vi "subSetItemInfoDependencies.vi"(8 "error in (no error)":errorcluster, 11 "SolutionBuilder in":refnum<class "SolutionBuilder.lvclass">) -> (0 "error out":errorcluster, 3 "SolutionBuilder out":refnum<class "SolutionBuilder.lvclass">)   [LabVIEW 2019, in "SolutionBuilder.lvlib" / "SolutionBuilder.lvclass"]
uses:
  SolutionBuilder.lvclass
  NamePathMap.ctl
  SolutionBuilder.lvclass/SolutionBuilder.ctl
  ProjectItem/ProjectItem.lvclass
  SolutionBuilder.lvlib
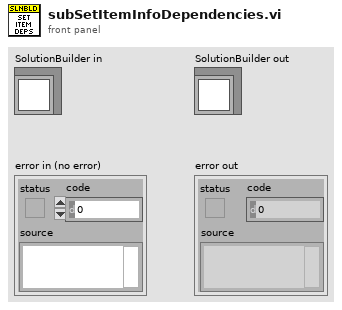
[diagram p1: front panel]
types:
  T1 = typedef "SolutionBuilder.lvlib/SolutionBuilder.lvclass/NamePathMap.ctl" = map{string, path}
  T2 = typedef "SolutionBuilder.lvlib/SolutionBuilder.lvclass/Hashes.ctl" = cluster{"Previous":T3, "Current":T3}
  T3 = typedef "SolutionBuilder.lvlib/SolutionBuilder.lvclass/HashMap.ctl" = map{T4, map{string, string}}
  T4 = typedef "SolutionBuilder.lvlib/SolutionBuilder.lvclass/IncrementalProjectInfo.ctl" = cluster{"Project path":string, "Build spec name":string, "Target":string}
  T5 = typedef "SolutionBuilder.lvlib/SolutionBuilder.lvclass/ProjectItemMap.ctl" = map{path, refnum<class "ProjectItem.lvclass">[]}
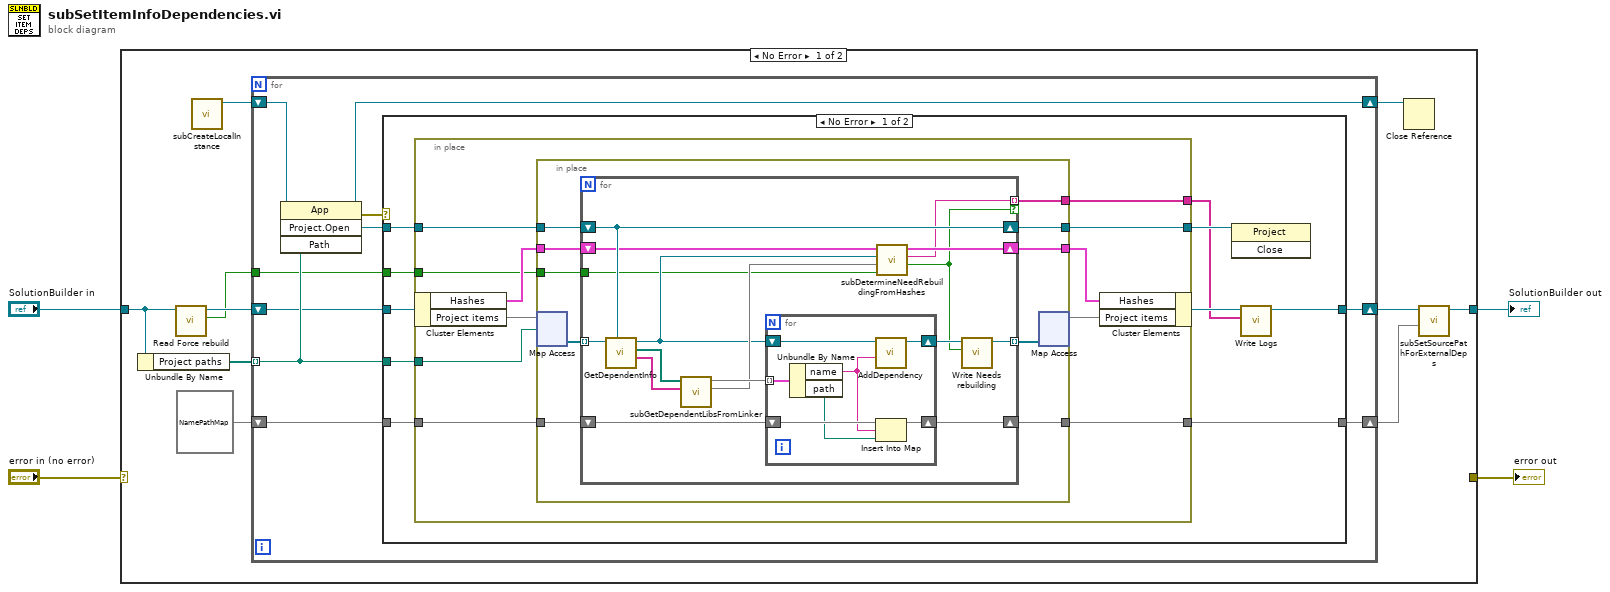
[diagram p0: block diagram]
diagram:
  n1 = case shown="No Error" "error in (no error)" {
    selector: "error in (no error)" -> [_ w81]
    tunnel: [w12 w82] -> w4
    tunnel: "SolutionBuilder in" -> [w7 w82]
    tunnel: [_ w81] -> w1
    frame No Error {
      n2 = Unbundle By Name(w7) -> ("Project paths"=w14:path[])
      n3 = call "Read Force rebuild.vi"("SolutionBuilder in"=w7) -> ("Force rebuild"=w5:bool, "SolutionBuilder out"=w6:refnum<class "SolutionBuilder.lvclass">)  [unwired: 9 in]
      n4 = call "subCreateLocalInstance.vi"() -> ("Application out"=w10:refnum<vi>)  [unwired: 11 in]
      n5 = for {
        tunnel: w14 -> [w22] mode=indexing
        shift-right: [w23] -> w13
        shift-left: T1 {} ("Dependency libs") -> [w24]
        shift-right: [w18] -> w9
        shift-left: w10 -> [w19]
        shift-right: [w16] -> w8
        shift-left: w6 -> [w17]
        tunnel: w5 -> [w15]
        n6 = invoke class="App" method="Project.Open"(reference=w19, "Path"=w22) -> (reference out=w18:refnum<vi>, error out=w21:errorcluster, "Project:Open"=w20:refnum<vi>)  [unwired: 2 in, 1 out]
        n7 = case shown="No Error" w21 {
          tunnel: w24 -> [w34 w80]
          tunnel: [w33 w80] -> w23
          tunnel: w22 -> [w32 _]
          tunnel: w20 -> [w31 _]
          tunnel: w17 -> [w29 w79]
          tunnel: [w27 w79] -> w16
          tunnel: w15 -> [w25 _]
          frame No Error {
            n8 = in-place {
              in-place-border: w34 -> [w45]
              in-place-border: [w44] -> w33
              in-place-border: w32 -> [w43]
              in-place-border: w31 -> [w42]
              in-place-border: [w41] -> w30
              in-place-border: [w36] -> w26
              in-place-border: w25 -> [w35]
              n9 = in-place-cluster #1(w29) -> ("Hashes"=w38:T2, "Project items"=w40:T5)
              n10 = in-place {
                in-place-border: [w53] -> w44
                in-place-border: w45 -> [w52]
                in-place-border: w42 -> [w51]
                in-place-border: [w50] -> w41
                in-place-border: w38 -> [w49]
                in-place-border: [w48] -> w37
                in-place-border: [w47] -> w36
                in-place-border: w35 -> [w46]
                n11 = in-place-map #2(w40, w43) -> (w55:refnum<class "ProjectItem.lvclass">[])  [unwired: 1 in, 1 out]
                n12 = for {
                  tunnel: w55 -> [w67] mode=indexing
                  tunnel: [w63] -> w54 mode=indexing
                  shift-right: [w71] -> w53
                  shift-left: w52 -> [w70]
                  shift-right: [w68] -> w50
                  shift-left: w51 -> [w68]
                  shift-right: [w61] -> w48
                  shift-left: w49 -> [w62]
                  tunnel: [w58] -> w47 mode=indexing if=w57
                  tunnel: w46 -> [w56]
                  n13 = call "GetDependentInfo.vi"("Project ref"=w68, "ProjectItem in"=w67) -> ("Dependent owning libs"=w65:string[], "Dependent paths"=w66:path[], "ProjectItem out"=w59:refnum<class "ProjectItem.lvclass">)  [unwired: 6 in, 1 out]
                  n14 = call "subGetDependentLibsFromLinker.vi"("Owning libs"=w65, "Paths"=w66) -> ("Dependency files"=w60:set{path}, "Dependency libs"=w69:T1)  [unwired: 8 in]
                  n15 = for {
                    tunnel: w69 -> [w74] mode=indexing
                    shift-right: [w77] -> w64
                    shift-left: w59 -> [w78]
                    shift-right: [w76] -> w71
                    shift-left: w70 -> [w75]
                    n16 = Unbundle By Name(w74) -> ("name"=w73:string, "path"=w72:path)
                    n17 = call "AddDependency.vi"("Dependency"=w73, "ProjectItem in"=w78) -> ("ProjectItem out"=w77:refnum<class "ProjectItem.lvclass">)  [unwired: 8 in, 1 out]
                    n18 = Insert Into Map(map in=w75, key=w73, value=w72) -> (map out=w76:T1)  [unwired: 2 out]
                  }
                  n19 = call "subDetermineNeedRebuildingFromHashes.vi"("Force rebuild"=w56, "Dependency files"=w60, "ProjectItem in"=w59, "Hashes in"=w62) -> ("Needs rebuilding"=w57:bool, "Log string"=w58:string, "Hashes out"=w61:T2)  [unwired: 5 in]
                  n20 = call "Write Needs rebuilding.vi"("Needs rebuilding"=w57, "ProjectItem in"=w64) -> ("ProjectItem out"=w63:refnum<class "ProjectItem.lvclass">)  [unwired: 9 in]
                }
                n21 = in-place-map #2(w54) -> (w39:T5)  [unwired: 1 in, 2 out]
              }
              n22 = in-place-cluster #1("Hashes"=w37, "Project items"=w39) -> (w28:refnum<class "SolutionBuilder.lvclass">)
            }
            n23 = invoke class="Project" method="Close"(reference=w30) -> ()  [unwired: 2 in, 3 out]
            n24 = call "Write Logs.vi"("Log entries"=w26, "SolutionBuilder in"=w28) -> ("SolutionBuilder out"=w27:refnum<class "SolutionBuilder.lvclass">)  [unwired: 9 in]
          }
          frame Error {
          }
        }
      }
      n25 = Close Reference(reference=w9) -> ()  [unwired: 1 in, 1 out]
      n26 = call "subSetSourcePathForExternalDeps.vi"("Dependency libs"=w13, "SolutionBuilder in"=w8) -> ("SolutionBuilder out"=w12:refnum<class "SolutionBuilder.lvclass">)  [unwired: 8 in, 1 out]
    }
    frame Error {
    }
  }
  "SolutionBuilder out" <- w4
  "error out" <- w1
